vi "Test Rotate String.vi"(8 "error in (no error)":errorcluster) -> (0 "error out":errorcluster, 3 "Pass?":bool)   [LabVIEW 2020]
uses:
  G-Unicode/Types/UTF-8 String/UTF-8 String.lvclass/UTF-8 String.ctl
  952276f3-5b34-4e34-8a1d-addec04de753.vi
  c633374f-98f1-4ebf-a8a9-694f055e3153.vi
  0ddb7cc8-26f8-44a6-9ae5-6ad694366a72.vi
  402b7c7c-7276-4835-8217-27b45ac813ca.vi
  b00df28f-3105-4a91-9dba-e25f43f45d63.vi
  G-Unicode/Private/Conversion/String as Encoded String.vi
  G-Unicode/Private/Conversion/Polymorphic VIs/String as Encoded String (LabVIEW String).vi
  G-Unicode/Private/Library/gu_rotate_string.vi
  c633374f-98f1-4ebf-a8a9-694f055e3153.vi/3a31b270-3bb6-4c58-a256-c5fcc2c98f09.vi
  c633374f-98f1-4ebf-a8a9-694f055e3153.vi/0ec5df2d-ef9b-4f84-a6a8-ffcedd45c4dc.vi
  G-Unicode/Private/Conversion/Polymorphic VIs/String as Encoded String (UTF-8 String).vi
  b00df28f-3105-4a91-9dba-e25f43f45d63.vi/3a31b270-3bb6-4c58-a256-c5fcc2c98f09.vi
  b00df28f-3105-4a91-9dba-e25f43f45d63.vi/0ec5df2d-ef9b-4f84-a6a8-ffcedd45c4dc.vi
  G-Unicode/Private/Conversion/Text to UTF-8.vi
  G-Unicode/Private/Conversion/Polymorphic VIs/Text to UTF-8 (LabVIEW String).vi
  G-Unicode/Private/Library/Result To Error.vi
  G-Unicode/Private/Conversion/Text as Encoded String.vi
  G-Unicode/Private/Conversion/Polymorphic VIs/Text as Encoded String (LabVIEW String).vi
  G-Unicode/Private/Conversion/Polymorphic VIs/Text as Encoded String (UTF-8 String).vi
  G-Unicode/Types/UTF-8 String/Read Encoded UTF-8 String.vi
  G-Unicode/Private/Library/gu_strlen.vi
  <vilib>/Utility/error.llb/Error Cluster From Error Code.vi
  G-Unicode/Types/UTF-8 String/UTF-8 String.lvclass
  a471ac35-12c8-4bfb-ae2f-202c5b1b399f.vi
  G-Unicode/Unicode/Controls/String Encoding.ctl
  G-Unicode/G-Unicode.lvlib
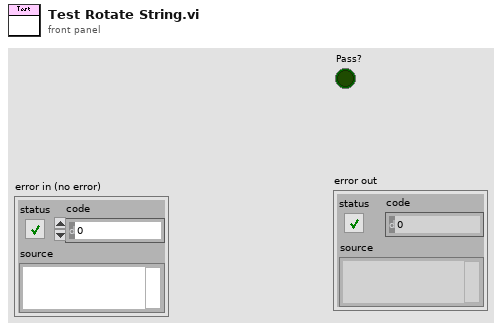
[diagram p1: front panel]
types:
  T1 = typedef "G-Unicode.lvlib/String Encoding.ctl" = enum16{"ANSI", "UTF-8", "UTF-16LE", "UTF-16BE", "Unknown"}
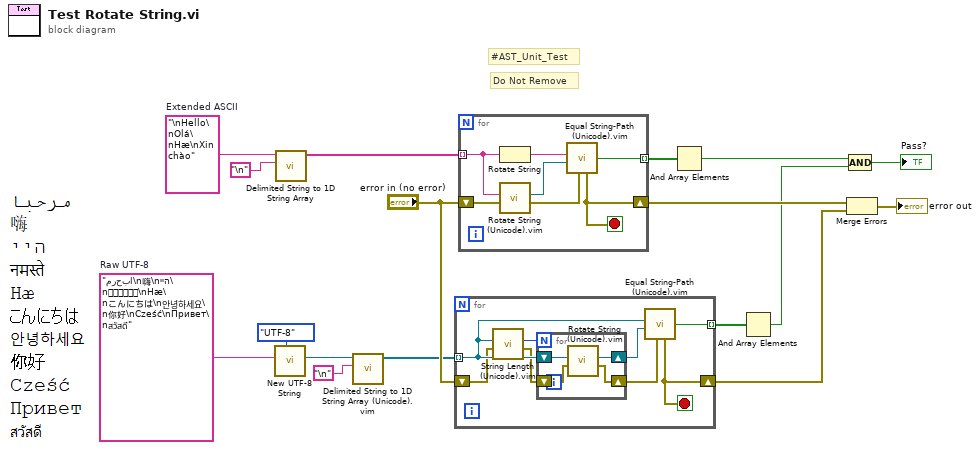
[diagram p0: block diagram]
diagram:
  w7 = "\nHello\nOlá\nHæ\nXin chào"  # Extended ASCII
  w2 = "مرحبا\n嗨\nהיי\nनमस्ते\nHæ\nこんにちは\n안녕하세요\n你好\nCześć\nПривет\nสวัสดี"  # Raw UTF-8
  # "Do Not Remove"
  # "#AST_Unit_Test"
  n1 = call "New UTF-8 String.vi"("Input Encoding (ANSI)"=String_Encoding."UTF-8", "String"=w2) -> ("UTF-8 String"=w4:refnum<class "UTF-8 String.lvclass">)  [unwired: 8 in, 1 out]
  n2 = call <vilib>:"Delimited String to 1D String Array.vi"("delimiter"="\n", "delimited string"=w7) -> ("string array"=w6:string[])  [unwired: 9 in]
  n3 = call "Delimited String to 1D String Array (Unicode).vim"("Delimiter (tab)"="\n", "Delimited String"=w4) -> ("String Array"=w1:refnum<class "UTF-8 String.lvclass">[])  [unwired: 8 in, 1 out]
  n4 = for {
    tunnel: w1 -> [w23] mode=indexing
    tunnel: [w25] -> w12 mode=indexing
    shift-right: [w18] -> w10
    shift-left: "error in (no error)" -> [w21]
    stop <- w18 stop-if-true
    n5 = call "String Length (Unicode).vim"("error in"=w21, "String"=w23) -> ("error out"=w20:errorcluster, "Length"=w22:i32)  [unwired: 8 in]
    n6 = for {
      N: w22 -> [_]
      shift-right: [w26] -> w19
      shift-left: w20 -> [w29]
      shift-right: [w27] -> w24
      shift-left: w23 -> [w28]
      n7 = call "Rotate String (Unicode).vim"("error in"=w29, "String"=w28) -> ("error out"=w26:errorcluster, "First Codepoint Last"=w27:refnum<class "UTF-8 String.lvclass">)  [unwired: 8 in]
    }
    n8 = call "Equal String-Path (Unicode).vim"("error in"=w19, "y"=w24, "x"=w23) -> ("error out"=w18:errorcluster, "Equal?"=w25:bool)  [unwired: 6 in]
  }
  n9 = for {
    tunnel: [w36] -> w14 mode=indexing
    shift-right: [w30] -> w17
    shift-left: "error in (no error)" -> [w34]
    tunnel: w6 -> [w35] mode=indexing
    stop <- w30 stop-if-true
    n10 = Rotate String(1:w35) -> (0:w33:string)
    n11 = call "Rotate String (Unicode).vim"("error in"=w34, "String"=w35) -> ("error out"=w31:errorcluster, "First Codepoint Last"=w32:refnum<class "UTF-8 String.lvclass">)  [unwired: 8 in]
    n12 = call "Equal String-Path (Unicode).vim"("error in"=w31, "y"=w32, "x"=w33) -> ("error out"=w30:errorcluster, "Equal?"=w36:bool)  [unwired: 6 in]
  }
  n13 = And Array Elements(Boolean array=w14) -> (logical AND=w13:bool)
  n14 = And Array Elements(Boolean array=w12) -> (logical AND=w11:bool)
  n15 = Merge Errors(w17, w10) -> (→"error out":errorcluster)
  n16 = Compound Arithmetic op=AND(w13, w11) -> (→"Pass?":bool)
